vi "VM Spy - MCListBox make row visible.vi"(6 "error in (no error)":errorcluster, 8 "visible row":i32, 9 "MCListbox Refnum":refnum<vi>) -> (0 "error out":errorcluster, 3 "dup MCListbox Refnum":refnum<vi>)   [LabVIEW 2021]
doc: "::: CalcExpress Toolkit :::\nCopyright (c) 2000-2026 Konstantin Shifershteyn. All rights reserved."
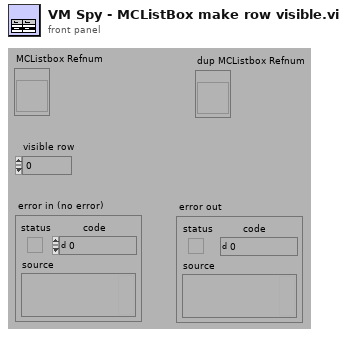
[diagram p1: front panel]
types:
  T1 = typedef "LVRowAndColumnUnsignedTypeDef.ctl" = cluster{"Row":u32, "Column":u32}
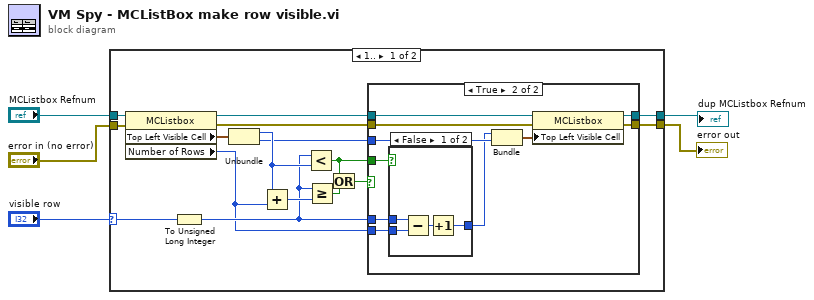
[diagram p0: block diagram]
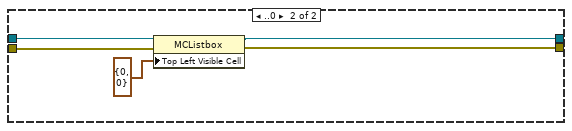
[diagram p4: hidden frame]
diagram:
  n1 = case shown="1.." "visible row" {
    selector: "visible row" -> [w14 _]
    tunnel: "MCListbox Refnum" -> [w21 w43]
    tunnel: [w17 w41] -> w3
    tunnel: [w16 w40] -> w2
    tunnel: "error in (no error)" -> [w15 w39]
    frame 1.. {
      n2 = property class="MCListbox"(reference=w21, error in=w15) -> (reference out=w19:refnum<vi>, error out=w18:errorcluster, "Top Left Visible Cell"=w20:T1, "Number of Rows"=w6:u32)
      n3 = To Unsigned Long Integer(number=w14) -> (unsigned 32bit integer=w7:u32)
      n4 = Unbundle(w20) -> ("Row"=w13:u32, "Column"=w9:u32)
      n5 = Add(x=w13, y=w6) -> (x+y=w12:u32)
      n6 = Less?(x=w7, y=w13) -> (x < y?=w8:bool)
      n7 = Greater Or Equal?(x=w7, y=w12) -> (x >= y?=w11:bool)
      n8 = Or(x=w8, y=w11) -> (x .or. y?=w10:bool)
      n9 = case shown="True" w10 {
        tunnel: w19 -> [w23 w32]
        tunnel: w18 -> [w22 w31]
        tunnel: [w23 w30] -> w17
        tunnel: [w22 w29] -> w16
        tunnel: w9 -> [_ w28]
        tunnel: w8 -> [_ w27]
        tunnel: w7 -> [_ w26]
        tunnel: w6 -> [_ w24]
        frame False {
        }
        frame True {
          n10 = case shown="False" w27 {
            tunnel: w26 -> [w37 w38]
            tunnel: [w34 w38] -> w25
            tunnel: w24 -> [w35 _]
            frame False {
              n11 = Subtract(x=w37, y=w35) -> (x-y=w36:u32)
              n12 = Increment(x=w36) -> (x+1=w34:u32)
            }
            frame True {
            }
          }
          n13 = Bundle(w25, "Column"=w28) -> (w33:cluster{u32, "Column":u32})  [unwired: 1 in]
          n14 = property class="MCListbox"(reference=w32, error in=w31, "Top Left Visible Cell"=w33) -> (reference out=w30:refnum<vi>, error out=w29:errorcluster)
        }
      }
    }
    frame ..0 {
      n15 = property class="MCListbox"(reference=w43, error in=w39, "Top Left Visible Cell"=cluster{u32, u32} {0, 0}) -> (reference out=w41:refnum<vi>, error out=w40:errorcluster)
    }
  }
  "dup MCListbox Refnum" <- w3
  "error out" <- w2
